vi "Prcess Data.vi"(8 "error in (no error)":errorcluster, 9 "Running":refnum<vi>, 10 "XY Plot":refnum<vi>, 11 "PG":refnum<class "Pressure Gain.lvclass">) -> (0 "error out":errorcluster, 3 "PG":refnum<class "Pressure Gain.lvclass">)   [LabVIEW 2025, in "Flow Grind.lvlib" / "Pressure Gain.lvclass"]
uses:
  Pressure Gain.lvclass
  Pressure Gain.lvclass/Pressure Gain.ctl
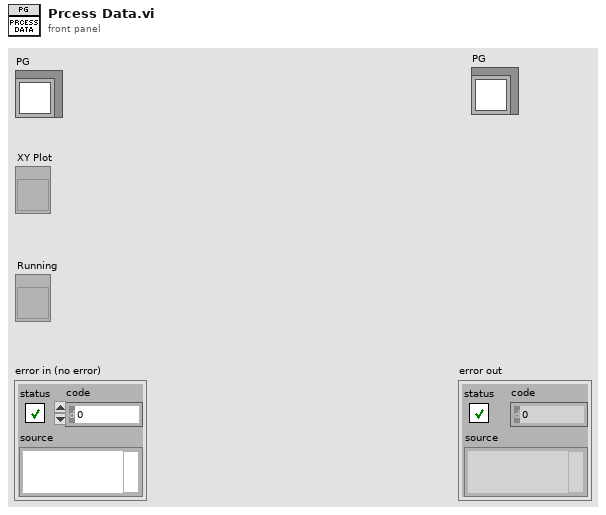
[diagram p1: front panel]
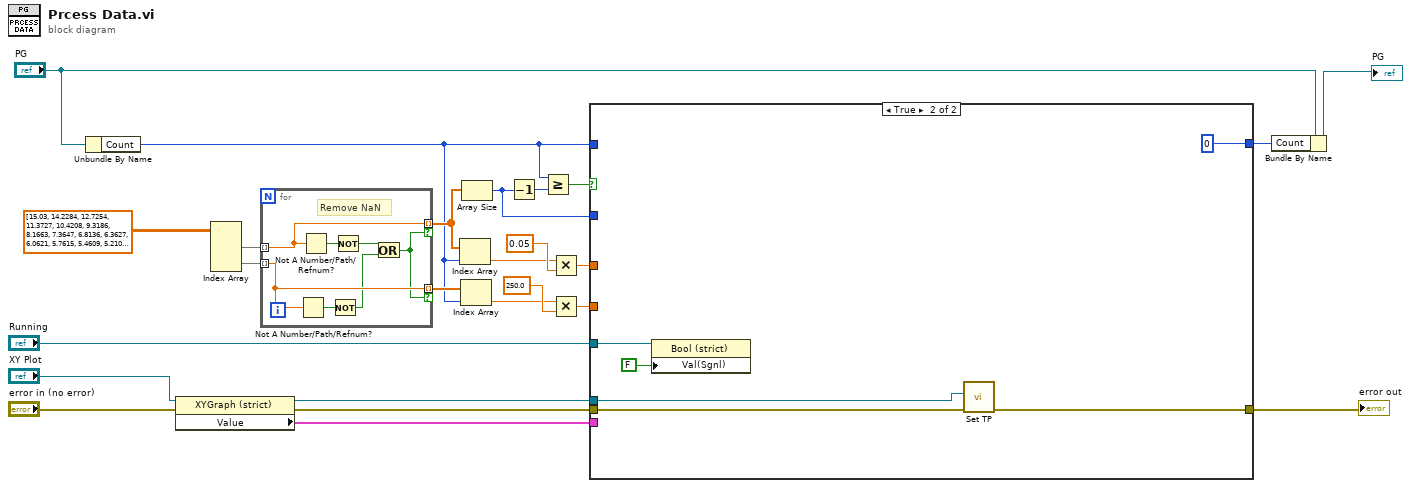
[diagram p0: block diagram]
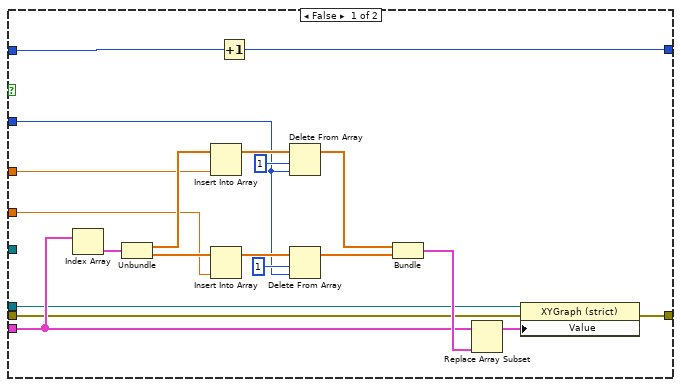
[diagram p2: hidden frame]
diagram:
  n1 = Unbundle By Name("PG") -> ("Count"=w12:i32)
  n2 = property class="XYGraph (strict)"(reference="XY Plot", error in="error in (no error)") -> (reference out=w13:refnum<vi>, error out=w17:errorcluster, "Value"=w16:cluster{dbl[], dbl[]}[])
  n3 = Index Array(array=dbl[][] [[15.03, 14.2284, 12.7254, 11.3727, 10.4208, 9.3186, 8.1663, 7.3647, 6.8136, 6.3627, 6.0621, 5.7615, 5.4609, 5.2104, 4.8597, 4.6593, 4.509, 4.3086, 4.0581, 3.8076, 3.507, 3.2565, 3.006, 2.7054, 2.5551, 2.3547, 2.2044, 2.0541, 1.8036, 1.5531, 1.3026, 1.002, 0.7515, 0.5511, 0.4008, 0.1002, -0.2004, -0.4008, -0.7515, -1.0521, -1.3527, -1.7034, -2.2044, -2.8557, -3.6573, -4.6092, -5.7114, -7.014, -8.016, -8.9178, -9.6693, -10.521, nan, nan, nan, nan, nan, nan, nan, nan, nan, nan, nan, nan, nan, nan, nan, nan], [-11.9357932, -11.8976187, -11.7757819, -11.5412005, -11.1747692, -10.5306628, -9.7025008, -8.9672438, -8.4006946, -7.9489022, -7.5837938, -7.2074985, -6.8413599, -6.4797298, -6.0220024, -5.6282905, -5.3575904, -5.0061417, -4.5881322, -4.1558815, -3.6121085, -3.0762002, -2.4234649, -1.7765761, -1.3145986, -0.8707762, -0.5146131, -0.1093126, 0.40181, 1.0005359, 1.6288074, 2.3084758, 2.8917529, 3.3778191, 3.8421829, 4.4080037, 4.9800247, 5.488318, 6.0848333, 6.7539309, 7.5044268, 8.4042368, 9.6903099, 10.9705643, 11.5684624, 11.781102, 11.8758014, 11.9254645, 11.9509021, 11.9683978, 11.9798972, 11.9903426, nan, nan, nan, nan, nan, nan, nan, nan, nan, nan, nan, nan, nan, nan, nan, nan], [0.0, 0.0, 0.0, 0.0, 0.0, 0.0, 0.0, 0.0, 0.0, 0.0, 0.0, 0.0, 0.0, 0.0, 0.0, 0.0, 0.0, 0.0, 0.0, 0.0, 0.0, 0.0, 0.0, 0.0, 0.0, 0.0, 0.0, 0.0, 0.0, 0.0, 0.0, 0.0, 0.0, 0.0, 0.0, 0.0, 0.0, 0.0, 0.0, 0.0, 0.0, 0.0, 0.0, 0.0, 0.0, 0.0, 0.0, 0.0, 0.0, 0.0, 0.0, 0.0, 0.0, 0.0, 0.0, 0.0, 0.0, 0.0, 0.0, 0.0, 0.0, 0.0, 0.0, 0.0, 0.0, 0.0, 0.0, 0.0], [0.0, 0.0, 0.0, 0.0, 0.0, 0.0, 0.0, 0.0, 0.0, 0.0, 0.0, 0.0, 0.0, 0.0, 0.0, 0.0, 0.0, 0.0, 0.0, 0.0, 0.0, 0.0, 0.0, 0.0, 0.0, 0.0, 0.0, 0.0, 0.0, 0.0, 0.0, 0.0, 0.0, 0.0, 0.0, 0.0, 0.0, 0.0, 0.0, 0.0, 0.0, 0.0, 0.0, 0.0, 0.0, 0.0, 0.0, 0.0, 0.0, 0.0, 0.0, 0.0, 0.0, 0.0, 0.0, 0.0, 0.0, 0.0, 0.0, 0.0, 0.0, 0.0, 0.0, 0.0, 0.0, 0.0, 0.0, 0.0]] ("array1")) -> (element #1=w25:dbl[], element #2=w24:dbl[])  [unwired: 4 in]
  n4 = for {
    tunnel: w25 -> [w32] mode=indexing
    tunnel: w24 -> [w29] mode=indexing
    tunnel: [w32] -> w21 mode=indexing if=w26
    tunnel: [w29] -> w23 mode=indexing if=w26
    # "Remove NaN"
    n5 = Not A Number/Path/Refnum?(number/path/refnum=w29) -> (NaN/Path/Refnum?=w30:bool)
    n6 = Not A Number/Path/Refnum?(number/path/refnum=w32) -> (NaN/Path/Refnum?=w31:bool)
    n7 = Not(x=w30) -> (.not. x?=w28:bool)
    n8 = Not(x=w31) -> (.not. x?=w27:bool)
    n9 = Or(x=w27, y=w28) -> (x .or. y?=w26:bool)
  }
  n10 = Index Array(array=w21, index=w12) -> (element=w2:dbl)
  n11 = Index Array(array=w23, index=w12) -> (element=w5:dbl)
  n12 = Array Size(array=w21) -> (size(s)=w11:i32)
  n13 = Decrement(x=w11) -> (x-1=w22:i32)
  n14 = Greater Or Equal?(x=w12, y=w22) -> (x >= y?=w20:bool)
  n15 = Multiply(x=w2, y=0.05 ("x")) -> (x*y=w1:dbl)
  n16 = Multiply(x=w5, y=250.0 ("x")) -> (x*y=w4:dbl)
  n17 = case shown="True" w20 {
    tunnel: w1 -> [w40 _]
    tunnel: w4 -> [w41 _]
    tunnel: w17 -> [w35 w55]
    tunnel: w16 -> [w42 _]
    tunnel: [w39 0] -> w14
    tunnel: w13 -> [w36 w53]
    tunnel: w12 -> [w38 _]
    tunnel: "Running" -> [_ w57]
    tunnel: w11 -> [w37 _]
    tunnel: [w33 w54] -> w10
    frame False {
      n18 = Index Array(array=w42) -> (element=w51:cluster{dbl[], dbl[]})  [unwired: 1 in]
      n19 = Unbundle(w51) -> (w49:dbl[], w50:dbl[])
      n20 = Insert Into Array(array=w49, new element=w40) -> (w46:dbl[])  [unwired: 1 in]
      n21 = Insert Into Array(array=w50, new element=w41) -> (w47:dbl[])  [unwired: 1 in]
      n22 = Increment(x=w38) -> (x+1=w39:i32)
      n23 = Delete From Array(array=w46, length=1, index=w37) -> (array with subset deleted=w44:dbl[])  [unwired: 1 out]
      n24 = Delete From Array(array=w47, length=1, index=w37) -> (array with subset deleted=w43:dbl[])  [unwired: 1 out]
      n25 = Bundle(w44, w43) -> (w52:cluster{dbl[], dbl[]})  [unwired: 1 in]
      n26 = Replace Array Subset(array=w42, new element=w52) -> (w34:cluster{dbl[], dbl[]}[])  [unwired: 1 in]
      n27 = property class="XYGraph (strict)"(reference=w36, error in=w35, "Value"=w34) -> (error out=w33:errorcluster)  [unwired: 1 out]
    }
    frame True {
      n28 = property class="Bool (strict)"(reference=w57, "Val(Sgnl)"=FALSE ("Value (Signaling)")) -> ()  [unwired: 1 in, 2 out]
      n29 = call "Set TP.vi"("error in (no error)"=w55, "Main"=w53) -> ("error out"=w54:errorcluster)  [unwired: 9 in]
    }
  }
  "error out" <- w10
  n30 = Bundle By Name(cluster="PG", "Count"=w14) -> (→"PG":refnum<class "Pressure Gain.lvclass">)
